vi "recovery_point__e7fff1c149.vi"(6 "Initial position in voltage":dbl, 7 "voltage to displacement constant":dbl, 8 "recovery phase":dbl, 9 "periods":dbl, 10 "frequency":dbl, 11 "Amplitude":dbl) -> (2 "sine wave":dbl format="%0.2f")   [LabVIEW 2023]
uses:
  <vilib>/ptbypt/NI_PtbyPt.lvlib
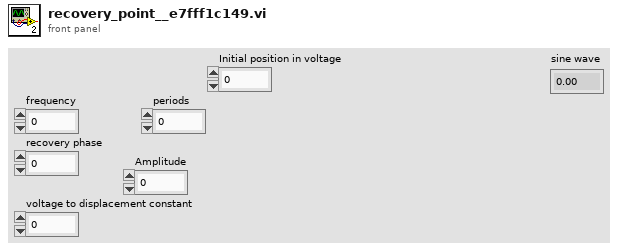
[diagram p1: front panel]
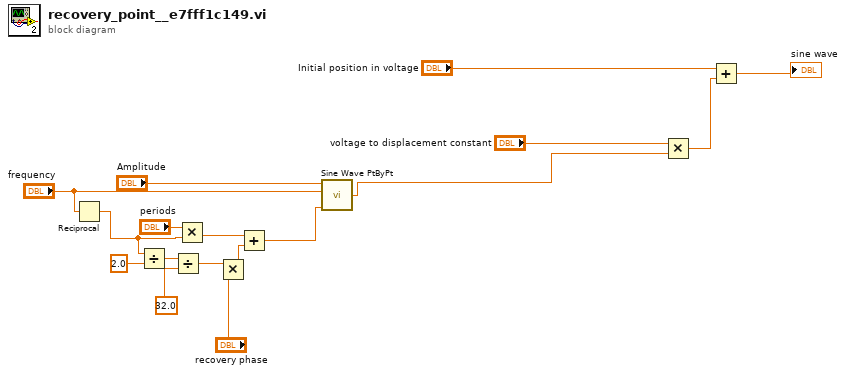
[diagram p0: block diagram]
diagram:
  n1 = Reciprocal(x="frequency") -> (1/x=w14:dbl)
  n2 = Divide(x=w14, y=2.0) -> (x/y=w12:dbl)
  n3 = Divide(x=w12, y=32.0) -> (x/y=w10:dbl)
  n4 = Multiply(x="periods", y=w14) -> (x*y=w7:dbl)
  n5 = Multiply(x=w10, y="recovery phase") -> (x*y=w8:dbl)
  n6 = Add(x=w7, y=w8) -> (x+y=w6:dbl)
  n7 = call <vilib>:"Sine Wave PtByPt.vi"("time"=w6, "frequency"="frequency", "amplitude"="Amplitude") -> ("sine wave"=w2:dbl)  [unwired: 1 in]
  n8 = Multiply(x="voltage to displacement constant", y=w2) -> (x*y=w3:dbl)
  n9 = Add(x="Initial position in voltage", y=w3) -> (x+y=→"sine wave":dbl)
